vi "Main.vi"() -> ()   [LabVIEW 2026]
doc: "Use this template to build a VI to use as a subVI."
panel:
  out "Last Update":string
  out "PLC Alive":bool
  in  "COM Port":refnum<visa-resource-name>
  in  "PLC Port":u16=5551
  in  "PLC Host":string="127.0.0.1"
  in  "PLC Transport":T1(ring)
  in  "Tab Control":T2(tab)
  out "Machine":picture
  out "PLC Connected":bool
  out "Auto Running":bool
  out "Manual Mode":bool
  out "Homed":bool
  out "Cycle Stopping":bool
  out "Alarm":bool
  out "E-Stop":bool
  out "Right Count":i32
  out "Left Count":i32
  out "Cycles":i32
  out "Alarm Code":i32
  out "Left Step":string
  out "Left Step ZH":string
  out "Home Step":string
  out "Home Step ZH":string
  out "Right Step":string
  out "Right Step ZH":string
  out "Alarm Text":string
  in  "Exit":bool
  out "Exit Status":string
  in  "Start":bool
  in  "Stop":bool
  in  "Home":bool
  in  "Reset":bool
  in  "Clear Counts":bool
  out "Manual Allowed":bool
  in  "L Forward":bool
  in  "L Rearward":bool
  in  "L Down":bool
  in  "L Up":bool
  in  "L Vacuum":bool
  in  "R Forward":bool
  in  "R Rearward":bool
  in  "R Down":bool
  in  "R Up":bool
  in  "R Vacuum":bool
  in  "Conveyors":bool
  in  "Write":bool
  in  "Vacuum Time (0.1 s)":u16=5
  in  "Release Time (0.1 s)":u16=5
  in  "Step Timeout (0.1 s)":u16=50
  in  "Target Cycles (0 = no limit)":u16
  out "X0 L gantry front pos":bool
  out "X1 L gantry rear pos":bool
  out "X2 R gantry front pos":bool
  out "X3 R gantry rear pos":bool
  out "X4 Front belt right end":bool
  out "X5 Rear belt left end":bool
  out "X6 L cylinder up":bool
  out "X7 L cylinder down":bool
  out "X10 Mode (ON auto)":bool
  out "X11 R cylinder up":bool
  out "X12 R cylinder down":bool
  out "X13 E-stop (NC)":bool
  out "X14 Not wired":bool
  out "X15 Not wired":bool
  out "X16 Not wired":bool
  out "X17 Not wired":bool
  out "Y0 L axis forward":bool
  out "Y1 L axis rearward":bool
  out "Y2 Conveyors run":bool
  out "Y3 R cylinder up":bool
  out "Y4 R cylinder down":bool
  out "Y5 Vacuum, both":bool
  out "Y6 R axis rearward":bool
  out "Y7 R axis forward":bool
  out "Y10 L down M8116":bool
  out "Y11 L up M8117":bool
  out "Y12 L vacuum (Y5)":bool
  out "Y13 Not wired":bool
  out "Y14 Not wired":bool
  out "Y15 Not wired":bool
  out "Y16 Not wired":bool
  out "Y17 Not wired":bool
  out "Alarm History":string[][](table)
  in  "Export CSV":bool
  # "ßB¾£ºTCP£½Ä£MÆ÷£¬RS-422£½C"
  # "Ä£”MÆ÷²ºÌ–"
  # "CÐòÁÐ²º"
  # "PLC 心跳有在變化"
  # "×îáá¸üÐÂ•rég"
  # "Åc PLC Í¨ÓÕý³£"
  # "ÓÒýˆéT°áß\\´Î”µ"
  # "×Ô„Óß\\ÞDÖÐ"
  # "×óýˆéT°áß\\´Î”µ"
  # "Ä£Ê½é_êPÔÚÊÖ„Ó"
  # "ÍêÕûÑ­­hÈ¦”µ"
  # "Ô­ücÍê³É"
  # "®³£´a 0£½Õý³£"
  # "Ñ­­hÍ£Ö¹ÖÐ"
  # "®³£ÖÐ"
  # "急停按下中"
  # "×óýˆéT²½Ðò"
  # "Ô­üc²½Ðò"
  # "ÓÒýˆéT²½Ðò"
  # "®³£ÕfÃ÷"
  # "†¢„Ó"
  # "ֹͣ"
  # "Ô­ücÍw"
  # "¡¾ß@ÊÇÊ²üN™CÌ¨¡¿ëpýˆéTÈ¡·ÅÑ­­h°áß\\™C\nƒÉ—lÆ½ÐÐ¡¢·½ÏòÏà·´µÄÝ”ËÍŽ§ÓÉÍ¬Ò»‚€Ý”³öòŒ„Ó£¬ƒÉ¶Ë¸÷¿çÒ»×ùýˆéT¡£\nÁ÷³Ì£ºÇ°Ý”ËÍŽ§£¨×ó¡úÓÒ£©ËÍµ½ÓÒ¶Ë ¡ú ÓÒýˆéTÎüÆð£¬°áµ½ááÝ”ËÍŽ§ ¡ú\n¡¡¡¡¡¡ááÝ”ËÍŽ§£¨ÓÒ¡ú×ó£©ËÍµ½×ó¶Ë ¡ú ×óýˆéTÎüÆð£¬·Å»ØÇ°Ý”ËÍŽ§£¬Ò»Ö±Ñ­­h¡£\nýˆéT™C˜‹£º™MÝS£½Ö±Á÷ñRß_£«ÂÝ—U£¬ÔÚÇ°‚È¡¢áá‚ÈÖ®égÒÆ„Ó£»\n¡¡¡¡¡¡¡¡¡¡Éý½µšâ¸×£½ëp„ÓëŠ´Åéy£»Îü±P£½Õæ¿Õ£¬†Î„Ó³£é]ëŠ´Åéy¡£\n¿ØÖÆ·Ö¹¤£ºFX3S PLC Ø“ØŸ„Ó×÷Åc»¥æi£¬±¾³ÌÊ½Ö»ÏÂÃüÁî¡¢¿´ î‘B¡¢¸Ä…¢”µ¡¢Ó›ä›¡£\n²Ù×÷í˜Ðò£ºHome »ØÔ­üc ¡ú ·Å¹¤¼þ ¡ú Start¡£Stop •þ×öÍêß@Ò»ÌË²ÅÍ£¡£"
  # "®³£Íw"
  # "計數清除"
  # "½YÊø³ÌÊ½"
  # "ÊÖÓÕfÃ÷£ºÄ£Ê½é_êP X10 ÇÐµ½ÊÖÓ£¨OFF£©¡¢]ÓÐ®³£¡¢Í¨ÓÕý³£r£¬×óßµÄô²ÅþÁÁ£¬°´âo²ÅÓÐÐ§¡£\nô²»ÁÁr°´ÁËÒ²²»þÓ£¬ß@ÊÇ PLC õÏÂíµÄ¡£"
  # "×óýˆéT£¨Ô­ücÔÚáá‚È£©"
  # "ÓÒýˆéT£¨Ô­ücÔÚÇ°‚È£©"
  # "上升（按住）"
  # "上升（按住）"
  # "往後（按住）"
  # "往前（按住）"
  # "往後（按住）"
  # "往前（按住）"
  # "下降（按住）"
  # "下降（按住）"
  # "Îü±P£¨°´Ò»ÏÂÇÐ“Q£©"
  # "Îü±P£¨°´Ò»ÏÂÇÐ“Q£©"
  # "ƒÉ—lÝ”ËÍŽ§£¨°´Ò»ÏÂÇÐ“Q£©"
  # "»¥æiÓÉ PLC ØØ£¬°´ÁË²»ÓÍ¨³£ÊÇ»¥æiõÏÂ£º\n1. â¸×²»ÔÚÉÏÏÞr£¬MÝS²»ÄÜÓ¡£¡¡2. ²»ÔÚÇ°È»òááÈ¶¨Î»ücr£¬â¸×²»ÄÜÏÂ½µ¡£\n3. ÍùÇ°£¯Íùáá¡¢ÉÏÉý£¯ÏÂ½µ²»þÍ¬rÓ×÷¡£¡¡4. Í¨ÓÖÐàr£¬ÊÖÓÓ×÷È«²¿×ÔÓÍ£Ö¹¡£\nÊÖÓÓß^CááþÇå³ýÔ­ücÍê³É£¬»Ø×ÔÓÇ°ÒªÔÙ°´Ò»´Î Home¡£"
  # "…¢”µÕfÃ÷£º¸ÄºÃ”µ×Öáá°´ Write ²Å•þŒ‘ßM PLC¡£†ÎÎ» 0.1 Ãë£¬ÀýÈç 5 £½ 0.5 Ãë¡£"
  # "Îü¸½•rég£¨D100£©£ºÎü±Pé_†¢ááµÈ¶à¾Ã²ÅÉÏÉý£¬Ì«¶Ì¿ÉÄÜÎü²»ÀÎ¡£¹ ‡ú 1¡«100"
  # "á·Årég£¨D101£©£ºÎü±PêPé]ááµÈ¶à¾Ã²ÅÉÏÉý£¬Ì«¶Ì¹¤¼þ¿ÉÄÜ±»§Æðí¡£¹ ú 1¡«100"
  # "Ó×÷Óâr£¨D102£©£ºÒ»Ó×÷³¬ß^ß@rég]µ½Î»¾Íó®³£¡£¹ ú 10¡«600"
  # "Ä¿˜ËÑ­­h´Î”µ£¨D103£©£º×öµ½ß@‚€È¦”µ×Ô„ÓÍ£Ö¹£¬0 £½ ²»ÏÞ¡£"
  # "Write£º°ÑÉÏÃæËÄ‚€ÖµŒ‘ßM PLC¡£"
  # "×¢Òâ£ºD100¡«D103 ”àëŠ²»±£³Ö£¬PLC ÖØÐÂÉÏëŠáá»Øµ½îAÔOÖµ£¬ÒªÔÙ°´Ò»´Î Write¡£"
  # "×óýˆéT_Ç°‚ÈÎ»ÖÃ"
  # "×ó™MÝS_ÍùÇ°"
  # "×óýˆéT_áá‚ÈÎ»ÖÃ"
  # "×ó™MÝS_Íùáá"
  # "ÓÒýˆéT_Ç°‚ÈÎ»ÖÃ"
  # "Ý”ËÍŽ§ß\\ÞD"
  # "ÓÒýˆéT_áá‚ÈÎ»ÖÃ"
  # "右氣缸_上升"
  # "前輸送帶_右端到位"
  # "右氣缸_下降"
  # "ááÝ”ËÍŽ§_×ó¶Ëµ½Î»"
  # "Îü±P_Õæ¿Õ(×óÓÒ¹²ÓÃ)"
  # "左氣缸_上限"
  # "ÓÒ™MÝS_Íùáá"
  # "左氣缸_下限"
  # "ÓÒ™MÝS_ÍùÇ°"
  # "模式(ON自動)"
  # "左氣缸_下降 M8116"
  # "右氣缸_上限"
  # "左氣缸_上升 M8117"
  # "右氣缸_下限"
  # "×óÎü±P(Y5)"
  # "急停(NC)"
  # "未接"
  # "未接"
  # "未接"
  # "未接"
  # "未接"
  # "未接"
  # "未接"
  # "未接"
  # "未接"
  # "…R³öµ½ logs\\alarm_export.csv£¨•þ¸²ÉwÅf™n£©¡£Ã¿ÈÕÍêÕû¼oä›ÔÚ logs\\yyyy-mm-dd.csv¡£"
  # "®³£´a¦ÕÕÅcÌÀí\n1¡¡¼±Í££º·Åé_¼±Í£ ¡ú Reset ¡ú Home\n10¡¡ÓÒMÝSÓâr£º²éñRß_¡¢X2¡¢X3¡¢OÏÞé_êP\n11¡¡ÓÒâ¸×Óâr£º²éâº¡¢X11¡¢X12\n20¡¡×óMÝSÓâr£º²éñRß_¡¢X0¡¢X1¡¢OÏÞé_êP\n21¡¡×óâ¸×Óâr£º²éâº¡¢X6¡¢X7\n30¡¡Ô­ücÍwÓâr£º²éÉÏÃæÈ«²¿\n40¡¡ÊÖÓÄ£Ê½Í¨ÓÖÐà£º²é 485 ¾ ¡ú Reset\n\nÍw£º°´Ò»´Î Reset Çå®³££¬ÔÙ°´Ò»´Î»ØÔ­üc¡£\n¼±Í£þ·Åµô¹¤¼þ£¬ÍwÇ°ÏÈ´_ÕJ¹¤¼þÎ»ÖÃ¡£"
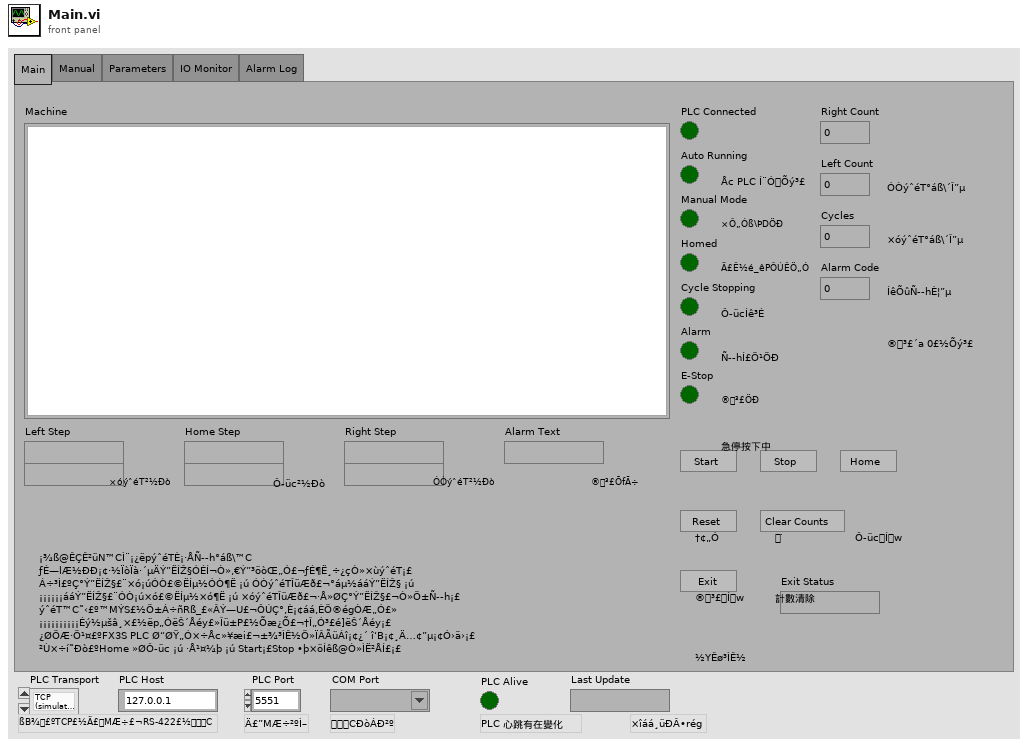
[diagram p1: front panel]
types:
  T1 = enum16{"TCP (simulator)", "RS-422 (COM)", "USB (COM)"}
  T2 = enum32{"Main", "Manual", "Parameters", "IO Monitor", "Alarm Log"}
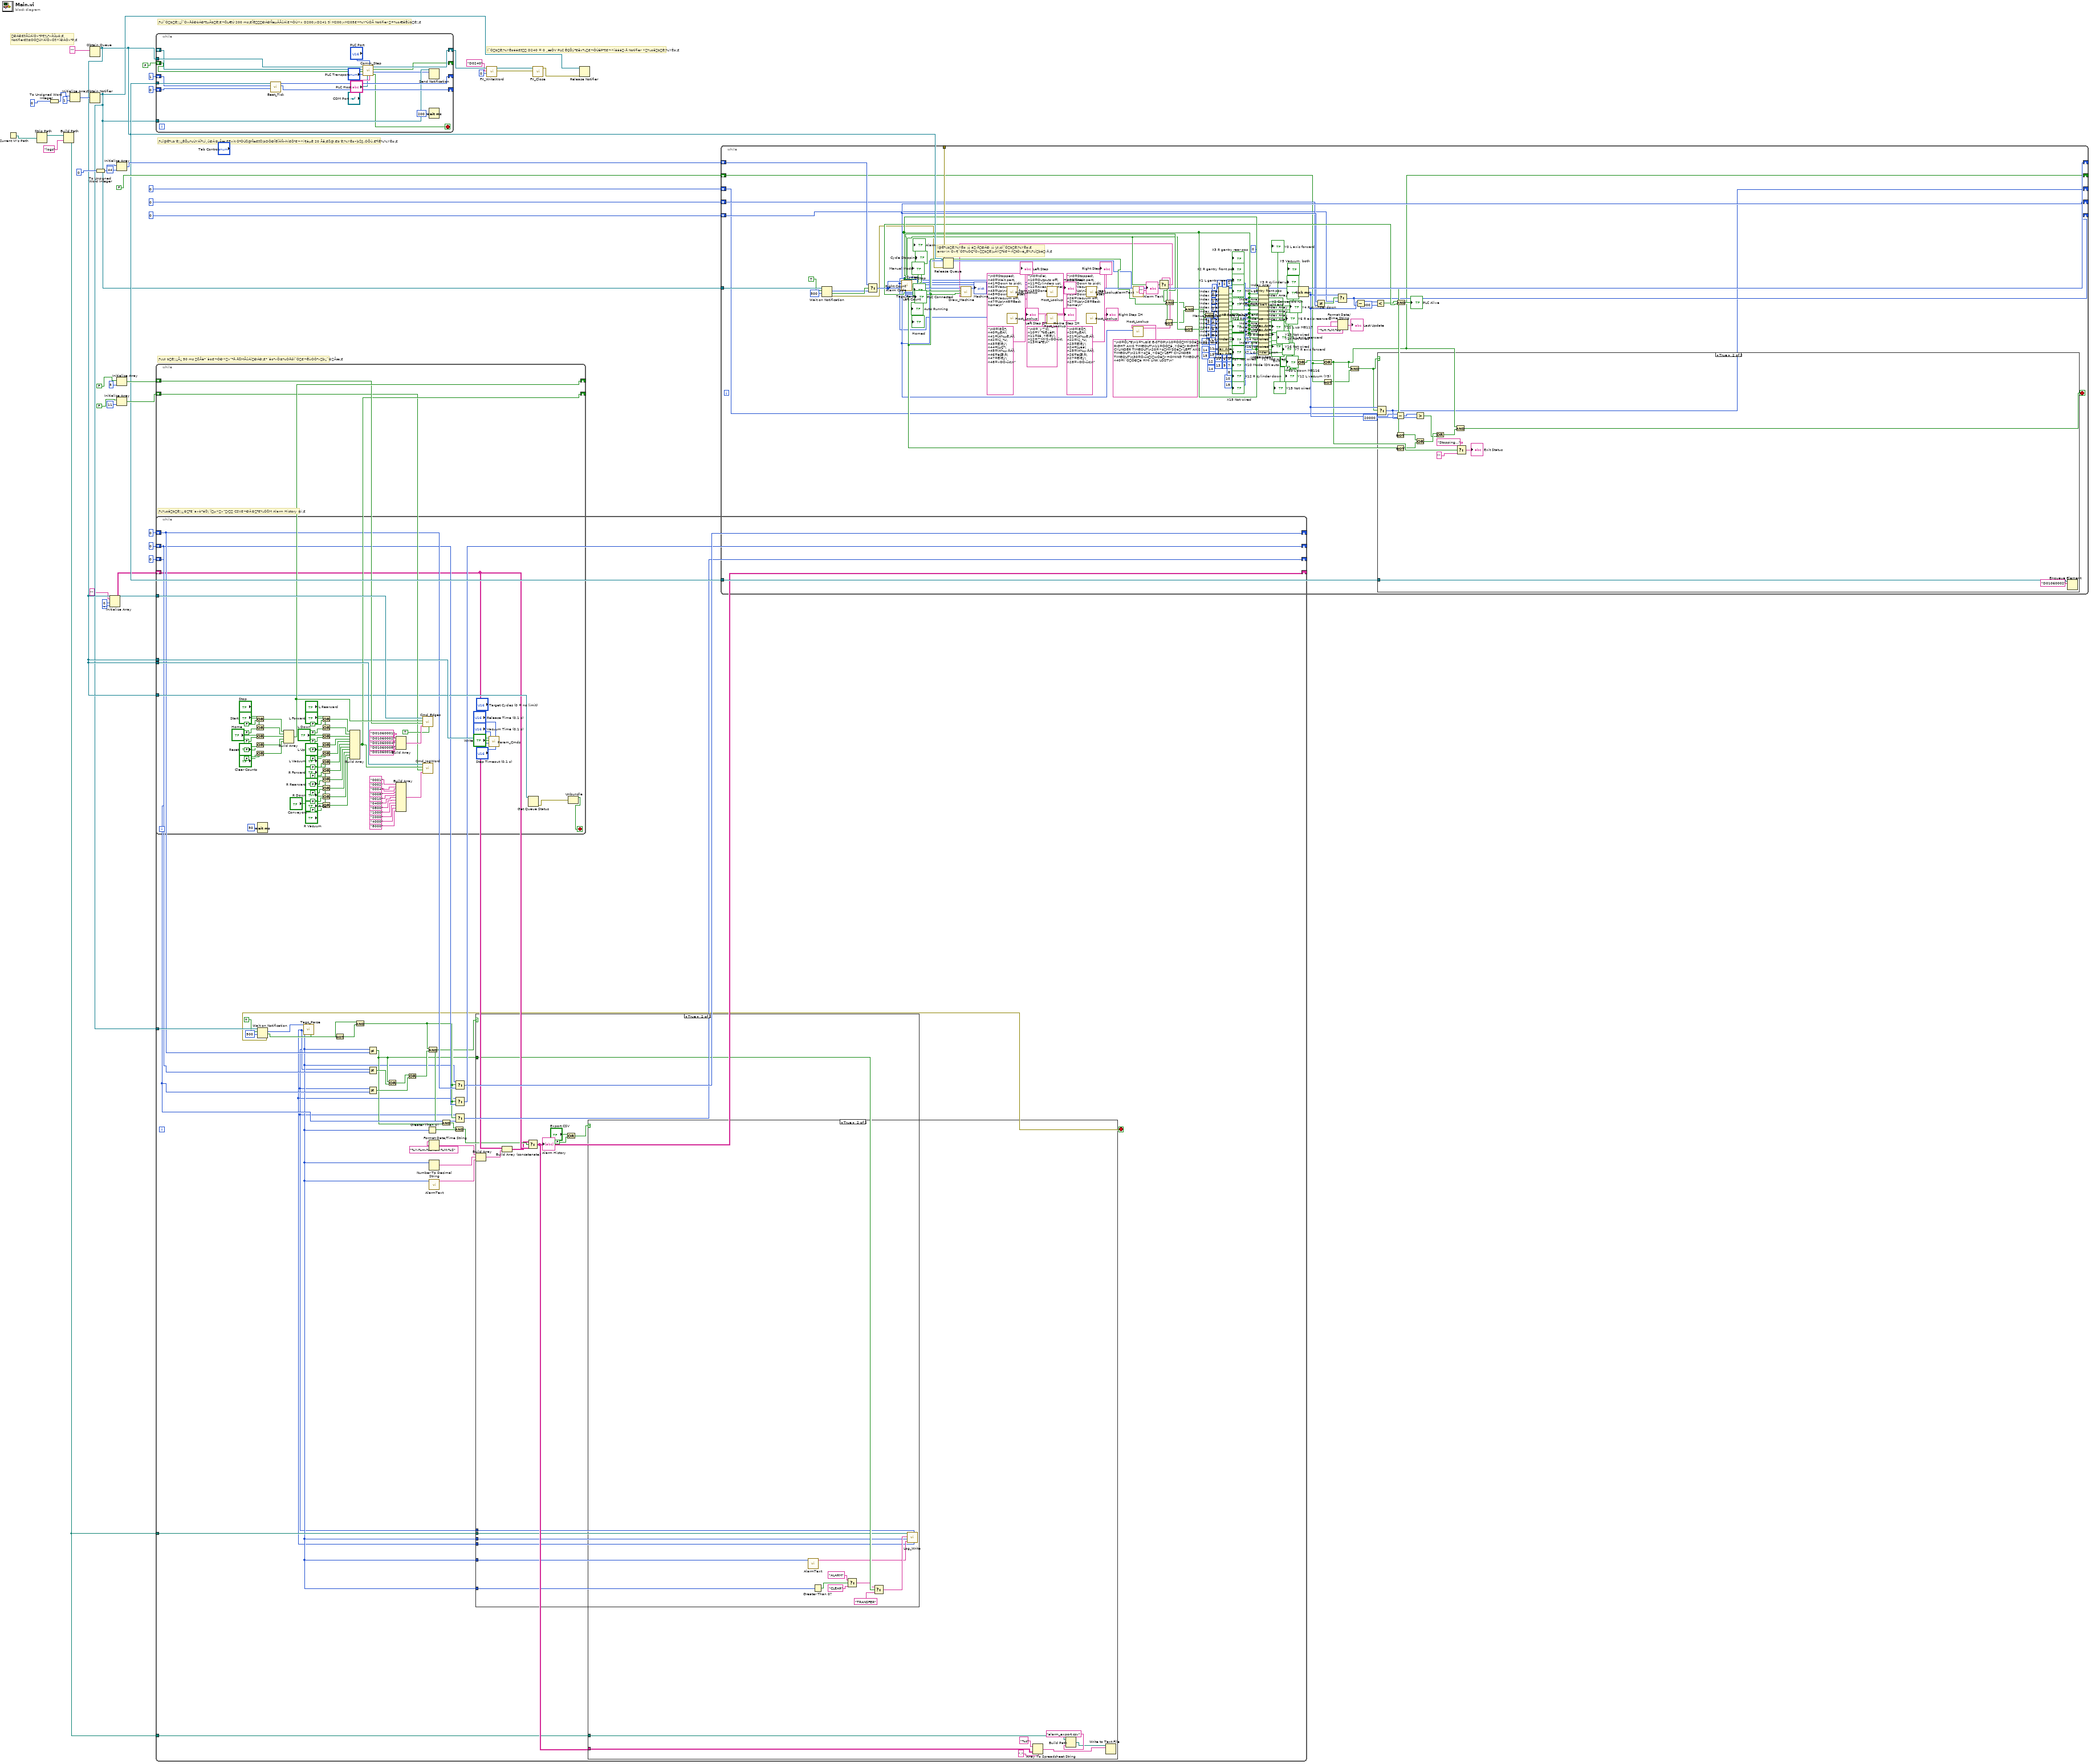
[diagram p0: block diagram]
diagram:
  # "ï@Ê¾ÞÈ¦½YÊø ¡ú á·ÅÐÁÐ ¡ú UI¡¢Í¨ÓÞÈ¦½YÊø¡£\nerror in Ò»¶¨Òª½ÓÇ°Ò»ÞÈ¦µÄÝ³ö£¬·ñtÒ»é_Ê¼¾Íþá·Å¡£"
  # "Í¨ÓÞÈ¦½YÊøáá£º D240 = 0 ¸æÔV PLC ÊÇÕý³£ëx¾£¬ÔÙêP²º£¬×îááá·Å Notifier ×¼oäÞÈ¦½YÊø¡£"
  # "ÐÁÐ£ºÃüÁîÒ»¹P¶¼²»ÄÜµô¡£\nNotifier£º±OÒÙYÁÏÖ»Òª×îÐÂÒ»¹P¡£"
  # "¡¾¼oäÞÈ¦¡¿®³£´a»ò°áß\\´Îµ×»¯r CSV£¬ÐÂ®³£¼ÓßM Alarm History ±í¡£"
  # "¡¾UI ÞÈ¦¡¿Ã¿ 50 ms ßÃè°´âo£¬ÓÐ×»¯²Å·ÅßMÃüÁîÐÁÐ¡£°´âo²»Ö±½ÓÅöÍ¨Ó£¬ËùÒÔ²»þ¿¨®Ãæ¡£"
  # "¡¾ï@Ê¾Þ’È¦¡¿ÊÕµ½ÙYÁÏ¾Í¸üÐÂ®‹Ãæ¡£Exit Ò²ÔÚß@Ñe£ºß\\ÞDÖÐÏÈÏÂÑ­­hÍ£Ö¹£¬×î¶àµÈ 20 Ãë¡£ß@‚€Þ’È¦½YÊø•þŽ§„ÓÕû‚€³ÌÊ½½YÊø¡£"
  # "¡¾Í¨ÓÞÈ¦¡¿Î¨Ò»ÅöÐòÁÐ²ºµÄÞÈ¦£¬ßLÆÚ 200 ms¡£ÏÈÐÁÐÑeµÄÃüÁî£¬ÔÙ×x D200¡«D241 ºÍ M200¡«M205£¬½Y¹ûÓÃ Notifier ÷½oÆäËûÞÈ¦¡£"
  n1 = Current VI's Path() -> (path=w37:path)
  n2 = Strip Path(path=w37) -> (stripped path=w36:path)  [unwired: 1 out]
  n3 = To Unsigned Word Integer(number=0) -> (unsigned 16bit integer=w39:u16)
  n4 = Build Path(base path=w36, name or relative path="logs") -> (appended path=w8:path)
  n5 = Initialize Array(w39, 1 ("dimension size")) -> (w38:u16[])
  n6 = Obtain Queue(element data type="") -> (queue out=w17:refnum<queue>)  [unwired: 4 in, 2 out]
  n7 = Obtain Notifier(notification data type=w38) -> (notifier out=w16:refnum<notifier>)  [unwired: 3 in, 2 out]
  n8 = To Unsigned Word Integer(number=0) -> (unsigned 16bit integer=w29:u16)
  n9 = Initialize Array("", 0 ("dimension size"), 0 ("dimension size")) -> (w9:string[][])
  n10 = Initialize Array(w29, 44 ("dimension size")) -> (w28:u16[])
  n11 = Initialize Array(FALSE, 5 ("dimension size")) -> (w21:bool[])
  n12 = Initialize Array(FALSE, 11 ("dimension size")) -> (w18:bool[])
  n13 = while {
    shift-right: [w52] -> w6
    shift-left: _ -> [w54]
    shift-right: [w51] -> _
    shift-left: FALSE -> [w53]
    shift-right: [w57] -> _
    shift-left: 1 ("Beat out") -> [w59]
    shift-right: [w56] -> _
    shift-left: u32 0 ("Last ms out") -> [w58]
    tunnel: w17 -> [w60]
    tunnel: w17 -> [w55]
    tunnel: w16 -> [w46]
    stop <- w43 stop-if-true
    n14 = call "Beat_Tick.vi"("Last ms"=w58, "Beat"=w59, "Queue"=w60) -> ("Last ms out"=w56:u32, "Beat out"=w57:i32)  [unwired: 7 in]
    n15 = call "Comm_Step.vi"("Host"="PLC Host", "Port"="PLC Port", "COM Port"="COM Port", "Transport"="PLC Transport", "Connected"=w53, "PLC Conn"=w54, "Queue"=w55) -> ("Stop"=w43:bool, "Words"=w45:u16[], "Connected out"=w51:bool, "PLC Conn out"=w52:refnum<visa-resource-name>)  [unwired: 1 in]
    n16 = Send Notification(notification=w45, notifier=w46) -> ()  [unwired: 1 in, 2 out]
    n17 = Wait (ms)(milliseconds to wait=u32 200) -> ()  [unwired: 1 out]
  }
  n18 = while {
    shift-right: [w93] -> _
    shift-left: w21 -> [w92]
    shift-right: [w83] -> _
    shift-left: w18 -> [w82]
    tunnel: w17 -> [w94]
    tunnel: w17 -> [w84]
    tunnel: w17 -> [w69]
    tunnel: w17 -> [w63]
    stop <- w61 stop-if-true
    n19 = Or(x="Start", y=FALSE) -> (x .or. y?=w132:bool)
    n20 = Or(x="Stop", y=FALSE) -> (x .or. y?=w131:bool)
    n21 = Or(x="Home", y=FALSE) -> (x .or. y?=w130:bool)
    n22 = Or(x="Reset", y=FALSE) -> (x .or. y?=w129:bool)
    n23 = Or(x="Clear Counts", y=FALSE) -> (x .or. y?=w128:bool)
    n24 = Wait (ms)(milliseconds to wait=u32 50) -> ()  [unwired: 1 out]
    n25 = Build Array(w132, w131, w130, w129, w128) -> (w93:bool[])
    n26 = Or(x="L Forward", y=FALSE) -> (x .or. y?=w105:bool)
    n27 = Or(x="L Rearward", y=FALSE) -> (x .or. y?=w104:bool)
    n28 = Or(x="L Down", y=FALSE) -> (x .or. y?=w103:bool)
    n29 = Or(x="L Up", y=FALSE) -> (x .or. y?=w102:bool)
    n30 = Or(x="L Vacuum", y=FALSE) -> (x .or. y?=w101:bool)
    n31 = Or(x="R Forward", y=FALSE) -> (x .or. y?=w100:bool)
    n32 = Or(x="R Rearward", y=FALSE) -> (x .or. y?=w99:bool)
    n33 = Or(x="R Down", y=FALSE) -> (x .or. y?=w98:bool)
    n34 = Or(x="R Up", y=FALSE) -> (x .or. y?=w97:bool)
    n35 = Or(x="R Vacuum", y=FALSE) -> (x .or. y?=w96:bool)
    n36 = Or(x="Conveyors", y=FALSE) -> (x .or. y?=w95:bool)
    n37 = Build Array(w105, w104, w103, w102, w101, w100, w99, w98, w97, w96, w95) -> (w83:bool[])
    n38 = Build Array("D01060001", "D01060002", "D01060004", "D01060008", "D01060010") -> (w86:string[])
    n39 = Build Array("0001", "0002", "0004", "0008", "0010", "0400", "0800", "1000", "2000", "4000", "8000") -> (w70:string[])
    n40 = call "Cmd_Edges.vi"("Rising Only"=TRUE, "Devices"=w86, "Prev"=w92, "Bits"=w93, "Queue"=w94) -> ()  [unwired: 7 in]
    n41 = call "Cmd_JogWord.vi"("Masks"=w70, "Prev"=w82, "Bits"=w83, "Queue"=w84) -> ()  [unwired: 8 in]
    n42 = call "Param_Cmds.vi"("Timeout"="Step Timeout (0.1 s)", "Target"="Target Cycles (0 = no limit)", "Release"="Release Time (0.1 s)", "Vacuum"="Vacuum Time (0.1 s)", "Write"="Write", "Queue"=w69) -> ()  [unwired: 6 in]
    n43 = Get Queue Status(queue=w63) -> (error out=w62:errorcluster)  [unwired: 2 in, 7 out]
    n44 = Unbundle(w62) -> ("status"=w61:bool)  [unwired: 2 out]
  }
  n45 = while {
    shift-right: [w168] -> _
    shift-left: 0 ("Alarm Code") -> [w176]
    shift-right: [w167] -> _
    shift-left: 0 ("Right Count") -> [w175]
    shift-right: [w166] -> _
    shift-left: 0 ("Left Count") -> [w174]
    shift-right: [w146] -> _
    shift-left: w9 -> [w153]
    tunnel: w16 -> [w183]
    tunnel: w8 -> [w163]
    tunnel: w8 -> [w145]
    stop <- w144 stop-if-true
    n46 = Wait on Notification(notifier=w183, ignore previous (F)=TRUE, timeout in ms (-1)=500) -> (notification=w180:u16[], timed out?=w179:bool, error out=w144:errorcluster)  [unwired: 1 in, 1 out]
    n47 = call "Tags_Parse.vi"("Words"=w180) -> ("Right Count"=w161:i32, "Left Count"=w160:i32, "Alarm Code"=w162:i32, "Connected"=w178:bool)  [unwired: 10 in, 13 out]
    n48 = Not(x=w179) -> (.not. x?=w177:bool)
    n49 = And(x=w178, y=w177) -> (x .and. y?=w170:bool)
    n50 = Not Equal?(x=w162, y=w176) -> (x != y?=w164:bool)
    n51 = Not Equal?(x=w161, y=w175) -> (x != y?=w173:bool)
    n52 = Not Equal?(x=w160, y=w174) -> (x != y?=w171:bool)
    n53 = Or(x=w164, y=w173) -> (x .or. y?=w172:bool)
    n54 = Or(x=w172, y=w171) -> (x .or. y?=w169:bool)
    n55 = Greater Than 0?(x=w162) -> (x > 0?=w158:bool)
    n56 = And(x=w170, y=w169) -> (x .and. y?=w165:bool)
    n57 = Format Date/Time String(time format string (%c)="%Y-%m-%d %H:%M:%S") -> (date/time string=w156:string)  [unwired: 2 in]
    n58 = Number To Decimal String(number=w162) -> (decimal integer string=w155:string)  [unwired: 1 in]
    n59 = call "AlarmText.vi"("Code"=w162) -> ("Text"=w154:string)  [unwired: 10 in]
    n60 = And(x=w165, y=w164) -> (x .and. y?=w159:bool)
    n61 = And(x=w159, y=w158) -> (x .and. y?=w151:bool)
    n62 = Select(t=w162, s=w170, f=w176) -> (s? t:f=w168:i32)
    n63 = Select(t=w161, s=w170, f=w175) -> (s? t:f=w167:i32)
    n64 = Select(t=w160, s=w170, f=w174) -> (s? t:f=w166:i32)
    n65 = case shown="True" w165 {
      tunnel: w162 -> [_ w204]
      tunnel: w162 -> [_ w203]
      tunnel: w164 -> [_ w199]
      tunnel: w163 -> [_ w196]
      tunnel: w162 -> [_ w194]
      tunnel: w161 -> [_ w192]
      tunnel: w160 -> [_ w191]
      frame False {
      }
      frame True {
        n66 = call "AlarmText.vi"("Code"=w204) -> ("Text"=w193:string)  [unwired: 10 in]
        n67 = Greater Than 0?(x=w203) -> (x > 0?=w202:bool)
        n68 = Select(t="ALARM", s=w202, f="CLEAR") -> (s? t:f=w198:string)
        n69 = Select(t=w198, s=w199, f="TRANSFER") -> (s? t:f=w195:string)
        n70 = call "Log_Write.vi"("Right Count"=w192, "Left Count"=w191, "Text"=w193, "Code"=w194, "Event"=w195, "Log Dir"=w196) -> ()  [unwired: 5 in, 1 out]
      }
    }
    n71 = Build Array(w156, w155, w154) -> (w152:string[])
    n72 = Build Array (concatenate)(w153, w152) -> (w150:string[][])
    n73 = Select(t=w150, s=w151, f=w153) -> (s? t:f=w146:string[][])
    "Alarm History" <- w146
    n74 = Or(x="Export CSV", y=FALSE) -> (x .or. y?=w147:bool)
    n75 = case shown="True" w147 {
      tunnel: w146 -> [_ w190]
      tunnel: w145 -> [_ w187]
      frame False {
      }
      frame True {
        n76 = Array To Spreadsheet String(delimiter (Tab)=",", array=w190, 3:"%s") -> (spreadsheet string=w184:string)
        n77 = Build Path(base path=w187, name or relative path="alarm_export.csv") -> (appended path=w185:path)
        n78 = Write to Text File(file (use dialog)=w185, text=w184) -> ()  [unwired: 2 in, 3 out]
      }
    }
  }
  n79 = call "FX_WriteWord.vi"("Value"=u16 0, "Device"="D0240", "PLC Conn"=w6) -> ("error out"=w2:errorcluster, "PLC Conn out"=w3:refnum<visa-resource-name>)  [unwired: 7 in]
  n80 = call "FX_Close.vi"("error in (no error)"=w2, "PLC Conn"=w3) -> ("error out"=w1:errorcluster)  [unwired: 9 in]
  n81 = Release Notifier(notifier=w16, error in (no error)=w1) -> ()  [unwired: 1 in, 3 out]
  n82 = while {
    shift-right: [w342] -> _
    shift-left: w28 -> [w344]
    shift-right: [w222] -> _
    shift-left: FALSE -> [w223]
    shift-right: [w217] -> _
    shift-left: u32 0 ("millisecond timer value") -> [w218]
    shift-right: [w238] -> _
    shift-left: 0 ("PLC Beat") -> [w237]
    shift-right: [w233] -> _
    shift-left: u32 0 ("millisecond timer value") -> [w234]
    tunnel: w16 -> [w348]
    tunnel: w17 -> [w219]
    tunnel: [w205] -> w7
    stop <- w209 stop-if-true
    n83 = Wait on Notification(notifier=w348, ignore previous (F)=TRUE, timeout in ms (-1)=500) -> (notification=w343:u16[], timed out?=w345:bool, error out=w205:errorcluster)  [unwired: 1 in, 1 out]
    n84 = Select(t=w344, s=w345, f=w343) -> (s? t:f=w342:u16[])
    n85 = call "Tags_Parse.vi"("Words"=w342) -> ("Right Step"=w316:i32, "Left Step"=w326:i32, "Home Step"=w321:i32, "Right Count"=→"Right Count":i32, "Left Count"=→"Left Count":i32, "Cycles"=→"Cycles":i32, "Alarm Code"=w328:i32, "PLC Beat"=w238:i32, "X"=w341:bool[], "Y"=w340:bool[], "Auto"=w337:bool, "Manual"=w336:bool, "Homed"=→"Homed":bool, "Alarm"=w333:bool, "E-Stop"=→"E-Stop":bool, "Cycle Stop"=→"Cycle Stopping":bool, "Connected"=w339:bool)  [unwired: 10 in]
    "PLC Connected" <- w339
    "Auto Running" <- w337
    "Manual Mode" <- w336
    "Alarm" <- w333
    "Alarm Code" <- w328
    n86 = call "Host_Lookup.vi"("Key"=w326, "Table"="\n0=Stopped\n40=Wait part\n41=Down to pick\n42=Vacuum on\n43=Up\n44=To front\n45=Down to place\n46=Vacuum off\n47=Up\n48=Back home\n") -> ("Text"=→"Left Step":string)  [unwired: 9 in]
    n87 = call "Host_Lookup.vi"("Key"=w326, "Table"="\n0=Í£Ö¹\n40=µÈÁÏ\n41=ÏÂ½µÈ¡ÁÏ\n42=Îü¸½\n43=ÉÏÉý\n44=ÍùÇ°\n45=ÏÂ½µ·ÅÁÏ\n46=áŒ·Å\n47=ÉÏÉý\n48=»ØÔ­üc\n") -> ("Text"=→"Left Step ZH":string)  [unwired: 9 in]
    n88 = call "Host_Lookup.vi"("Key"=w321, "Table"="\n0=Idle\n10=Outputs off\n11=Cylinders up\n12=Axes to home\n13=Done\n") -> ("Text"=→"Home Step":string)  [unwired: 9 in]
    n89 = call "Host_Lookup.vi"("Key"=w321, "Table"="\n0=´ý™C\n10=Ý”³öÈ«êP\n11=šâ¸×ÉÏÉý\n12=™MÝS»ØÔ­üc\n13=Íê³É\n") -> ("Text"=→"Home Step ZH":string)  [unwired: 9 in]
    n90 = call "Host_Lookup.vi"("Key"=w316, "Table"="\n0=Stopped\n20=Wait part\n21=Down to pick\n22=Vacuum on\n23=Up\n24=To rear\n25=Down to place\n26=Vacuum off\n27=Up\n28=Back home\n") -> ("Text"=→"Right Step":string)  [unwired: 9 in]
    n91 = call "Host_Lookup.vi"("Key"=w316, "Table"="\n0=Í£Ö¹\n20=µÈÁÏ\n21=ÏÂ½µÈ¡ÁÏ\n22=Îü¸½\n23=ÉÏÉý\n24=Íùáá\n25=ÏÂ½µ·ÅÁÏ\n26=áŒ·Å\n27=ÉÏÉý\n28=»ØÔ­üc\n") -> ("Text"=→"Right Step ZH":string)  [unwired: 9 in]
    n92 = call "AlarmText.vi"("Code"=w328) -> ("Text"=→"Alarm Text":string)  [unwired: 10 in]
    n93 = call "Host_Lookup.vi"("Key"=w328, "Table"="\n0=Õý³£\n1=¼±Í£ E-STOP\n10=ÓÒMÝSÓâr RIGHT AXIS TIMEOUT\n11=ÓÒâ¸×Óâr RIGHT CYLINDER TIMEOUT\n20=×óMÝSÓâr LEFT AXIS TIMEOUT\n21=×óâ¸×Óâr LEFT CYLINDER TIMEOUT\n30=Ô­ücÍwÓâr HOMING TIMEOUT\n40=Í¨ÓÖÐà HMI LINK LOST\n") -> ("Text"=w310:string)  [unwired: 9 in]
    n94 = Select(t=w310, s=w333, f="") -> (s? t:f=w308:string)
    n95 = call "Draw_Machine.vi"("Banner"=w308, "Connected"=w339, "Y"=w340, "X"=w341) -> ("Machine"=→"Machine":picture)  [unwired: 7 in]
    n96 = Not(x=w337) -> (.not. x?=w306:bool)
    n97 = And(x=w336, y=w339) -> (x .and. y?=w307:bool)
    n98 = Not(x=w333) -> (.not. x?=w304:bool)
    n99 = And(x=w307, y=w306) -> (x .and. y?=w305:bool)
    n100 = And(x=w305, y=w304) -> (x .and. y?=→"Manual Allowed":bool)
    n101 = Index Array(array=w341, index=0) -> (element=→"X0 L gantry front pos":bool)
    n102 = Index Array(array=w341, index=1) -> (element=→"X1 L gantry rear pos":bool)
    n103 = Index Array(array=w341, index=2) -> (element=→"X2 R gantry front pos":bool)
    n104 = Index Array(array=w341, index=3) -> (element=→"X3 R gantry rear pos":bool)
    n105 = Index Array(array=w341, index=4) -> (element=→"X4 Front belt right end":bool)
    n106 = Index Array(array=w341, index=5) -> (element=→"X5 Rear belt left end":bool)
    n107 = Index Array(array=w341, index=6) -> (element=→"X6 L cylinder up":bool)
    n108 = Index Array(array=w341, index=7) -> (element=→"X7 L cylinder down":bool)
    n109 = Index Array(array=w341, index=8) -> (element=→"X10 Mode (ON auto)":bool)
    n110 = Index Array(array=w341, index=9) -> (element=→"X11 R cylinder up":bool)
    n111 = Index Array(array=w341, index=10) -> (element=→"X12 R cylinder down":bool)
    n112 = Index Array(array=w341, index=11) -> (element=→"X13 E-stop (NC)":bool)
    n113 = Index Array(array=w341, index=12) -> (element=→"X14 Not wired":bool)
    n114 = Index Array(array=w341, index=13) -> (element=→"X15 Not wired":bool)
    n115 = Index Array(array=w341, index=14) -> (element=→"X16 Not wired":bool)
    n116 = Index Array(array=w341, index=15) -> (element=→"X17 Not wired":bool)
    n117 = Index Array(array=w340, index=0) -> (element=→"Y0 L axis forward":bool)
    n118 = Index Array(array=w340, index=1) -> (element=→"Y1 L axis rearward":bool)
    n119 = Index Array(array=w340, index=2) -> (element=→"Y2 Conveyors run":bool)
    n120 = Index Array(array=w340, index=3) -> (element=→"Y3 R cylinder up":bool)
    n121 = Index Array(array=w340, index=4) -> (element=→"Y4 R cylinder down":bool)
    n122 = Index Array(array=w340, index=5) -> (element=→"Y5 Vacuum, both":bool)
    n123 = Index Array(array=w340, index=6) -> (element=→"Y6 R axis rearward":bool)
    n124 = Index Array(array=w340, index=7) -> (element=→"Y7 R axis forward":bool)
    n125 = Index Array(array=w340, index=8) -> (element=→"Y10 L down M8116":bool)
    n126 = Index Array(array=w340, index=9) -> (element=→"Y11 L up M8117":bool)
    n127 = Index Array(array=w340, index=10) -> (element=→"Y12 L vacuum (Y5)":bool)
    n128 = Index Array(array=w340, index=11) -> (element=→"Y13 Not wired":bool)
    n129 = Index Array(array=w340, index=12) -> (element=→"Y14 Not wired":bool)
    n130 = Index Array(array=w340, index=13) -> (element=→"Y15 Not wired":bool)
    n131 = Index Array(array=w340, index=14) -> (element=→"Y16 Not wired":bool)
    n132 = Index Array(array=w340, index=15) -> (element=→"Y17 Not wired":bool)
    n133 = Or(x="Exit", y=FALSE) -> (x .or. y?=w224:bool)
    n134 = Tick Count (ms)() -> (millisecond timer value=w235:u32)
    n135 = Not Equal?(x=w238, y=w237) -> (x != y?=w236:bool)
    n136 = Or(x=w224, y=w223) -> (x .or. y?=w222:bool)
    n137 = Not(x=w223) -> (.not. x?=w221:bool)
    n138 = Select(t=w235, s=w236, f=w234) -> (s? t:f=w233:u32)
    n139 = Format Date/Time String(time format string (%c)="%H:%M:%S") -> (date/time string=→"Last Update":string)  [unwired: 2 in]
    n140 = And(x=w222, y=w221) -> (x .and. y?=w220:bool)
    n141 = Subtract(x=w235, y=w233) -> (x-y=w232:u32)
    n142 = Less?(x=w232, y=u32 3000) -> (x < y?=w230:bool)
    n143 = Select(t=w235, s=w220, f=w218) -> (s? t:f=w217:u32)
    n144 = case shown="True" w220 {
      tunnel: w219 -> [_ w350]
      frame False {
      }
      frame True {
        n145 = Enqueue Element(queue=w350, element="D01060002") -> ()  [unwired: 2 in, 3 out]
      }
    }
    n146 = Subtract(x=w235, y=w217) -> (x-y=w216:u32)
    n147 = Not(x=w337) -> (.not. x?=w214:bool)
    n148 = Not(x=w339) -> (.not. x?=w213:bool)
    n149 = And(x=w230, y=w339) -> (x .and. y?=→"PLC Alive":bool)
    n150 = Greater?(x=w216, y=u32 20000) -> (0:w211:bool)
    n151 = Or(x=w214, y=w213) -> (x .or. y?=w212:bool)
    n152 = Or(x=w212, y=w211) -> (x .or. y?=w210:bool)
    n153 = And(x=w222, y=w210) -> (x .and. y?=w209:bool)
    n154 = Select(t="Stopping...", s=w222, f="") -> (s? t:f=→"Exit Status":string)
  }
  n155 = Release Queue(queue=w17, error in (no error)=w7) -> ()  [unwired: 1 in, 3 out]
